vi "Set use unicode and default Lang.vi"(8 "Default Language":i32, 9 "Startup Language":i32, 11 "Obj.":T1={"Type"=enum."Caption", "Translation ANSI"=[], "Translation Unicode"=[]}) -> (1 "Translation out":string, 2 "Unicode?":bool)   [LabVIEW 2019, in "Language Selection.lvlib"]
doc: "Sets the translation language and checks if the output translation language belongs to Unicode or ANSI character set.\n\nIf the input translation is empty, the control will be translated to the default language.\n- - -\nCopyright (c) 2026, Merecs Engineering GmbH"
uses:
  Language Selection.lvlib
  TypeDefs/Cluster PropertyTranslation.ctl
  TypeDefs/Enum Property Type.ctl
panel:
  # "Connector Pane"
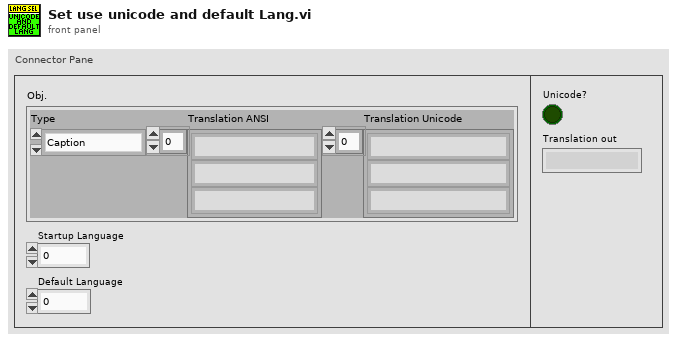
[diagram p1: front panel]
types:
  T1 = typedef "Language Selection.lvlib/Cluster PropertyTranslation.ctl" = cluster{"Type":T2, "Translation ANSI":string[], "Translation Unicode":string[]}
  T2 = typedef "Language Selection.lvlib/Enum Property Type.ctl" = enum16{"NA", "Caption", "String Value", "Boolean Text", "Ring Strings", "1D Array Elements", "2D Array Elements", "(MC)Listbox Header", "(MC)Listbox Items", "Tab Pages Names", "X & Y GraphChart", "Plot Names", "Table Headers", "Table Items", "TipStrip", "Combobox Strings", "Cursor Name", "Tree Col Headers"}
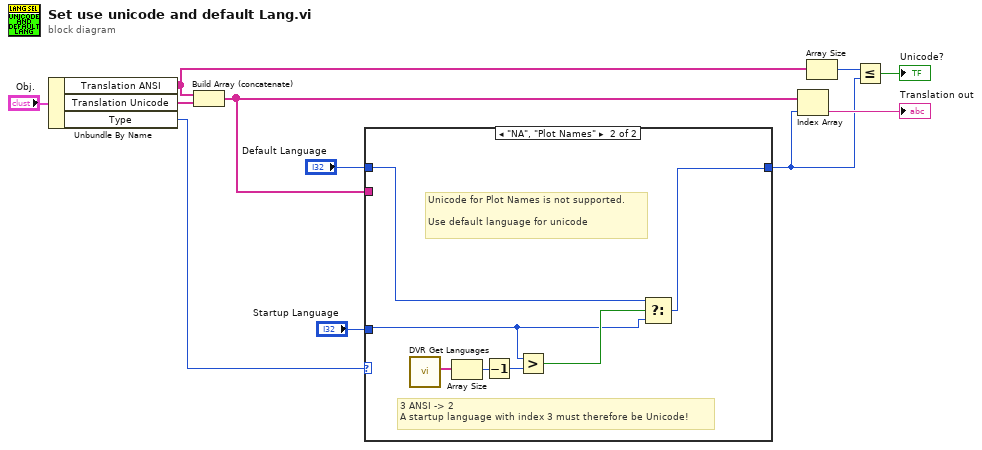
[diagram p0: block diagram]
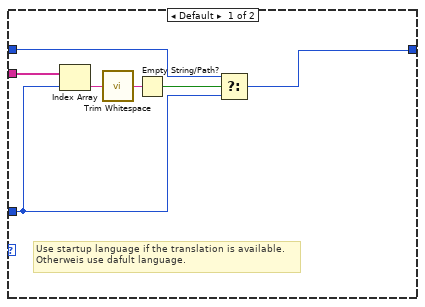
[diagram p2: hidden frame]
diagram:
  n1 = Unbundle By Name("Obj.") -> ("Translation ANSI"=w7:string[], "Translation Unicode"=w6:string[], "Type"=w1:T2)
  n2 = Build Array (concatenate)(w7, w6) -> (w3:string[])
  n3 = case shown="\"NA\", \"Plot Names\"" w1 {
    tunnel: "Startup Language" -> [w13 w22]
    tunnel: "Default Language" -> [w15 w20]
    tunnel: w3 -> [w14 _]
    tunnel: [w12 w21] -> w2
    frame Default {
      # "Use startup language if the translation is available.\nOtherweis use dafult language."
      n4 = Index Array(array=w14, index=w13) -> (element=w16:string)
      n5 = call <vilib>:"Trim Whitespace.vi"("string"=w16) -> ("trimmed string"=w17:string)  [unwired: 1 in]
      n6 = Empty String/Path?(string/path=w17) -> (empty?=w18:bool)
      n7 = Select(t=w15, s=w18, f=w13) -> (s? t:f=w12:i32)
    }
    frame "NA", "Plot Names" {
      # "3 ANSI -> 2\nA startup language with index 3 must therefore be Unicode!"
      # "Unicode for Plot Names is not supported.\n\nUse default language for unicode"
      n8 = call "DVR Get Languages.vi"() -> ("ANSI"=w25:string[])  [unwired: 8 in, 3 out]
      n9 = Array Size(array=w25) -> (size(s)=w24:i32)
      n10 = Decrement(x=w24) -> (x-1=w19:i32)
      n11 = Greater?(x=w22, y=w19) -> (0:w23:bool)
      n12 = Select(t=w20, s=w23, f=w22) -> (s? t:f=w21:i32)
    }
  }
  n13 = Index Array(array=w3, index=w2) -> (element=→"Translation out":string)
  n14 = Array Size(array=w7) -> (size(s)=w10:i32)
  n15 = Less Or Equal?(x=w10, y=w2) -> (x <= y?=→"Unicode?":bool)
